vi "Target ID Map.vi"(8 "error in (no error)":errorcluster, 11 "Cluster in":refnum<class "Cluster Config.lvclass">) -> (0 "error out":errorcluster, 2 "Target ID Map":map{string, T1}(c390), 3 "Cluster out":refnum<class "Cluster Config.lvclass">)   [LabVIEW 2020, in "VolatusConfig.lvlib" / "Cluster Config.lvclass"]
uses:
  Cluster Config.lvclass
  C:/dev/lv20CE/relink/lv-volatus/VolatusConfig/VolatusConfigElement/VolatusConfigElement.lvclass
  Target Info.ctl
  Target Type.ctl
  Meta Type.ctl
  VolatusConfigElement/VolatusConfigElement.lvclass/VolatusConfigElement.ctl
  VolatusConfigElement/Element.vi
  Node/Node Config.lvclass
  lv-cdm/CDM-Config/Config Lookup/Match Meta.vi
  lv-cdm/CDM-Config/Config Element/Owner.vi
  lv-cdm/CDM-Config/Config Manager/Lookup Descendant.vi
  lv-cdm/CDM-Config/Config Filter/Config Lookup.lvclass
  Cluster Config.lvclass/Cluster Config.ctl
  VolatusConfigElement/VolatusConfigElement.lvclass
  VolatusConfig.lvlib
  lv-cdm/CDM-Config/Config Element/Config Element.lvclass
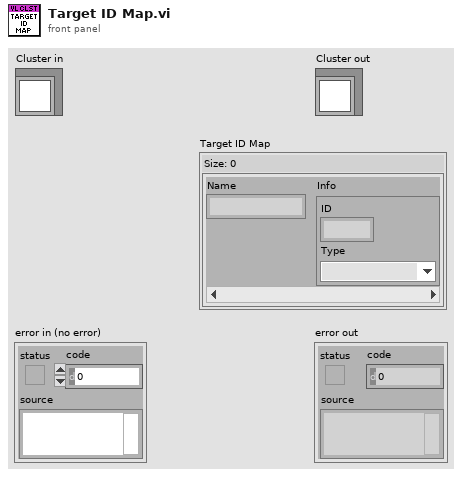
[diagram p1: front panel]
types:
  T1 = typedef "VolatusConfig.lvlib/Target Info.ctl" = cluster{"ID":u32, "Type":T2}
  T2 = typedef "VolatusConfig.lvlib/Target Type.ctl" = enum16{"Unknown", "Node", "Group"}
  T3 = typedef "VolatusConfig.lvlib/Meta Type.ctl" = enum16{"UNKNOWN", "VL_System", "VL_Cluster", "VL_Node", "VL_Task", "VL_Group", "VL_Channel", "VL_Task_List", "VL_Scaling", "VL_Sensor", "VL_Sensor_List", "VL_Scale"}
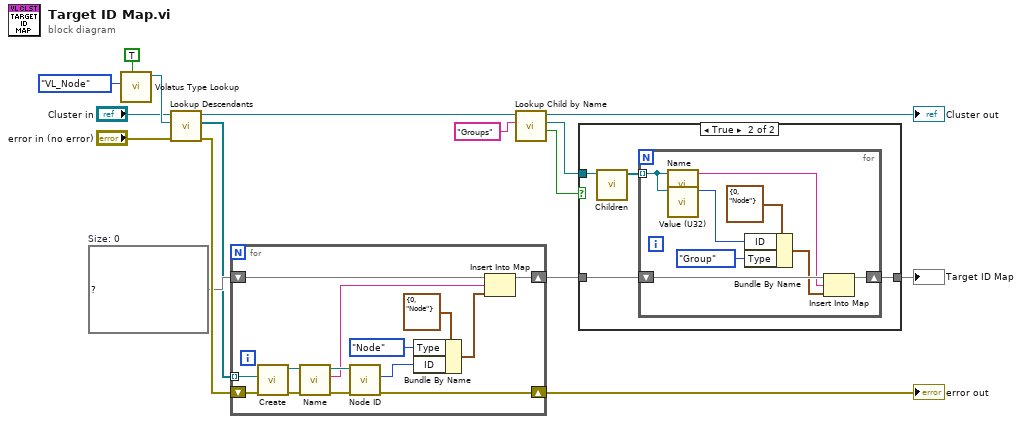
[diagram p0: block diagram]
diagram:
  w12 = map{string, T1} {}  # Size: 0
  n1 = call "Volatus Type Lookup.vi"("Don't Recurse Past Match (F)"=TRUE, "Meta Type"=Meta_Type."VL_Node") -> ("Config Lookup out"=w14:refnum<class "Config Lookup.lvclass">)  [unwired: 8 in, 1 out]
  n2 = call "Lookup Descendants.vi"("error in (no error)"="error in (no error)", "Lookup"=w14, "VolatusConfigElement in"="Cluster in") -> ("error out"=w16:errorcluster, "Descendants"=w11:refnum<class "Config Element.lvclass">[], "VolatusConfigElement out"=w8:refnum<class "Cluster Config.lvclass">)  [unwired: 6 in]
  n3 = for {
    shift-right: [w21] -> w3
    shift-left: w12 -> [w24]
    tunnel: w11 -> [w30] mode=indexing
    shift-right: [w22] -> w7
    shift-left: w16 -> [w28]
    n4 = call "Create.vi"("error in (no error)"=w28, "Element"=w30) -> ("error out"=w27:errorcluster, "Node out"=w29:refnum<class "Node Config.lvclass">)  [unwired: 8 in]
    n5 = call "Name.vi"("error in (no error)"=w27, "VolatusConfigElement in"=w29) -> ("error out"=w25:errorcluster, "Name"=w23:string, "VolatusConfigElement out"=w26:refnum<class "Node Config.lvclass">)  [unwired: 7 in]
    n6 = call "Node ID.vi"("error in (no error)"=w25, "Node in"=w26) -> ("error out"=w22:errorcluster, "Node ID"=w19:u32)  [unwired: 7 in, 1 out]
    n7 = Bundle By Name(cluster=T1 {"ID"=0, "Type"=enum."Node"} ("Target Info"), "Type"=Target_Type."Node", "ID"=w19) -> (w17:T1)
    n8 = Insert Into Map(map in=w24, key=w23, value=w17) -> (map out=w21:map{string, T1})  [unwired: 2 out]
  }
  "error out" <- w7
  n9 = call "Lookup Child by Name.vi"("Child Name"="Groups", "VolatusConfigElement in"=w8) -> ("Found"=w4:bool, "Child"=w2:refnum<class "Config Element.lvclass">, "VolatusConfigElement out"=→"Cluster out":refnum<class "Cluster Config.lvclass">)  [unwired: 6 in, 1 out]
  n10 = case shown="True" w4 {
    tunnel: w3 -> [w31 w33]
    tunnel: w2 -> [_ w35]
    tunnel: [w31 w32] -> w1
    frame False {
      # "Specifying target groups is optional."
    }
    frame True {
      n11 = call "Children.vi"("Config Element in"=w35) -> ("Elements"=w34:refnum<class "Config Element.lvclass">[])  [unwired: 9 in, 1 out]
      n12 = for {
        tunnel: w34 -> [w43] mode=indexing
        shift-right: [w40] -> w32
        shift-left: w33 -> [w42]
        n13 = call "Name.vi"("Config Element in"=w43) -> ("Name"=w41:string)  [unwired: 9 in, 1 out]
        n14 = call "Value (U32).vi"("Config Element in"=w43) -> ("U32 Value"=w37:u32)  [unwired: 9 in, 1 out]
        n15 = Bundle By Name(cluster=T1 {"ID"=0, "Type"=enum."Node"} ("Target Info"), "ID"=w37, "Type"=Target_Type."Group") -> (w36:T1)
        n16 = Insert Into Map(map in=w42, key=w41, value=w36) -> (map out=w40:map{string, T1})  [unwired: 2 out]
      }
    }
  }
  "Target ID Map" <- w1
